vi "Lire config Pt.vi"(2 "error in (no error)":errorcluster caption="entrée d'erreur (pas d'erreur)", 3 "refnum":T1) -> (0 "error out":errorcluster caption="sortie d'erreur", 1 "refnum out":T1 caption="refnum en sortie")   [LabVIEW 2022 SP3]
uses:
  <vilib>/Utility/config.llb/Config Data RefNum.ctl
  <vilib>/Utility/config.llb/Read Key (String).vi
  Variables globales/Variable glob Pt.vi
  <vilib>/Utility/config.llb/Read Key (I32).vi
  <vilib>/Utility/config.llb/Read Key (Boolean).vi
  <vilib>/Utility/config.llb/NI_LVConfig.lvlib
panel:
  out "Nombre de modules":i32=1 min=1
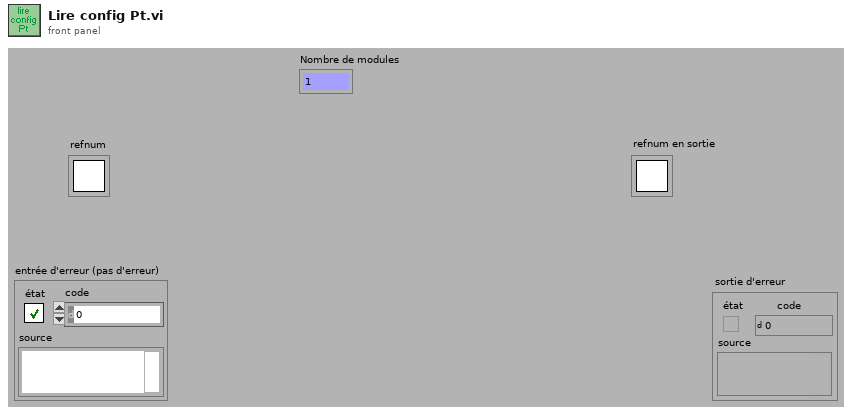
[diagram p1: front panel]
types:
  T1 = typedef "NI_LVConfig.lvlib/Config Data RefNum.ctl" = refnum<k1>
  T2 = cluster{"Nom tache Pt":refnum<k21>, "Noms des Pt":string[], "Nb Pt":i16, "Sélection Pt":bool[], "Nom Pt sélectionnées":string[]}[]
  T3 = cluster{"Nom tache Pt":refnum<k21>, "Noms des Pt":string[], "Nb Pt":i16, "Selection Pt":bool[], "Nom Pt selectionnees":string[]}[]
  T4 = cluster{"Nom tache Pt":refnum<k21>, "Noms des Pt":string[], "Nb Pt":i16, "Selection Pt":bool[], "Nom Pt selectionnees":string[]}
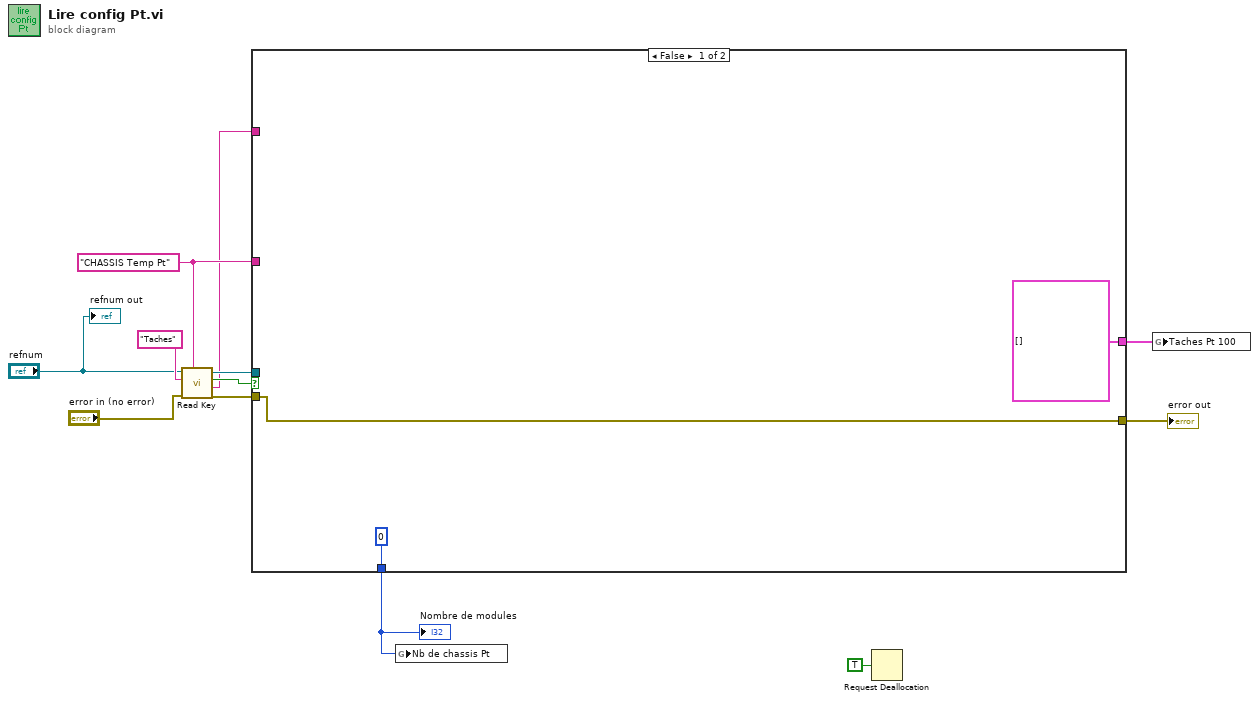
[diagram p0: block diagram]
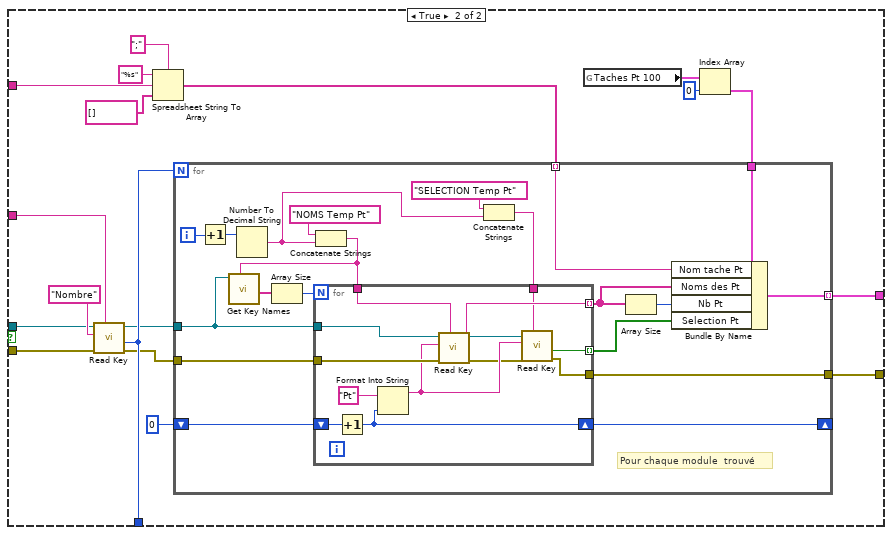
[diagram p2: hidden frame]
diagram:
  w11 = "CHASSIS Temp Pt" ("section")
  n1 = call-poly <vilib>:"Read Key.vi"("section"=w11, "error in (no error)"="error in (no error)", "key"="Taches", "refnum"="refnum") -> ("error out"=w8:errorcluster, "value"=w2:string, "found?"=w5:bool, "refnum out"=w7:T1)  [unwired: 4 in]
  n2 = case shown="False" w5 {
    tunnel: [w14 w33] -> w12
    tunnel: w11 -> [_ w27]
    tunnel: [0 ("value") w32] -> w10
    tunnel: w8 -> [w14 w30]
    tunnel: w7 -> [_ w29]
    tunnel: [T2 [] w21] -> w3
    tunnel: w2 -> [_ w17]
    frame False {
    }
    frame True {
      n3 = call-poly <vilib>:"Read Key.vi"("section"=w27, "error in (no error)"=w30, "key"="Nombre", "refnum"=w29) -> ("error out"=w25:errorcluster, "value"=w32:i32, "refnum out"=w26:T1)  [unwired: 4 in, 1 out]
      n4 = Spreadsheet String To Array(delimiter (Tab)=";" ("séparateur (Tabulation)"), format string="%s" ("chaîne de format"), spreadsheet string=w17, array type (2D Dbl)=string[] [] ("type de tableau (2D de dbl)")) -> (array=w16:string[])
      n5 = global read "Variable glob Pt.vi" "Taches Pt 100"() -> (w24:T3)
      n6 = Index Array(array=w24, index=0 ("indice")) -> (element=w22:T4)
      n7 = for {
        N: w32 -> [_]
        tunnel: [w53] -> w33
        tunnel: w26 -> [w43]
        tunnel: w25 -> [w52]
        shift-right: [w48] -> _
        shift-left: 0 -> [w49]
        tunnel: w22 -> [w39]
        tunnel: [w37] -> w21 mode=indexing
        tunnel: w16 -> [w34] mode=indexing
        i -> [w51]
        # "Pour chaque module  trouvé"
        n8 = Increment(x=w51) -> (x+1=w50:i32)
        n9 = Number To Decimal String(number=w50) -> (decimal integer string=w40:string)  [unwired: 1 in]
        n10 = Concatenate Strings("NOMS Temp Pt" ("chaîne initiale"), w40) -> (w41:string)
        n11 = call <vilib>:"Get Key Names.vi"("section"=w41, "refnum"=w43) -> ("key names"=w44:string[])  [unwired: 6 in, 3 out]
        n12 = Array Size(array=w44) -> (size(s)=w42:i32)
        n13 = Concatenate Strings("SELECTION Temp Pt" ("chaîne initiale"), w40) -> (w45:string)
        n14 = for {
          N: w42 -> [_]
          tunnel: w43 -> [w66]
          tunnel: w52 -> [w65]
          tunnel: [w61] -> w36 mode=indexing
          tunnel: [w63] -> w38 mode=indexing
          tunnel: [w62] -> w53
          shift-right: [w59] -> w48
          shift-left: w49 -> [w60]
          tunnel: w41 -> [w58]
          tunnel: w45 -> [w57]
          n15 = Increment(x=w60) -> (x+1=w59:i32)
          n16 = Format Into String(initial string="Pt" ("chaîne initiale"), w59) -> (resulting string=w56:string)  [unwired: 2 in, 1 out]
          n17 = call-poly <vilib>:"Read Key.vi"("section"=w58, "error in (no error)"=w65, "key"=w56, "refnum"=w66) -> ("error out"=w55:errorcluster, "value"=w61:string, "refnum out"=w54:T1)  [unwired: 4 in, 1 out]
          n18 = call-poly <vilib>:"Read Key.vi"("section"=w57, "error in (no error)"=w55, "key"=w56, "refnum"=w54) -> ("error out"=w62:errorcluster, "value"=w63:bool)  [unwired: 4 in, 2 out]
        }
        n19 = Array Size(array=w36) -> (size(s)=w35:i32)
        n20 = Bundle By Name(cluster=w39, "Nom tache Pt"=w34, "Noms des Pt"=w36, "Nb Pt"=w35, "Selection Pt"=w38) -> (w37:T4)
      }
    }
  }
  "error out" <- w12
  "Nombre de modules" <- w10
  n21 = global write "Variable glob Pt.vi" "Nb de chassis Pt"(w10) -> ()
  n22 = Request Deallocation(TRUE ("flag")) -> ()
  n23 = global write "Variable glob Pt.vi" "Taches Pt 100"(w3) -> ()
  "refnum out" <- "refnum"
